vi "Calculate Analog and Digital Channel Values.vi"(8 "Use Default Values":bool=TRUE, 9 "Execute Sequence":bool=TRUE, 10 "current time":timestamp, 11 "Settings in":T1) -> (0 "Digital Values to Write":bool[](array[boolean]), 1 "Analog Values to Write":dbl[](array[numeric]), 2 "Sequence State Channels to Write":dbl[](array[numeric]), 3 "Settings out":T1)   [LabVIEW 2020, in "Sequencer with Output Values.lvlib" / "Sequencer with Output Values.lvclass"]
uses:
  Sequencer with Output Values.lvclass
  Params.ctl
  Step Settings.ctl
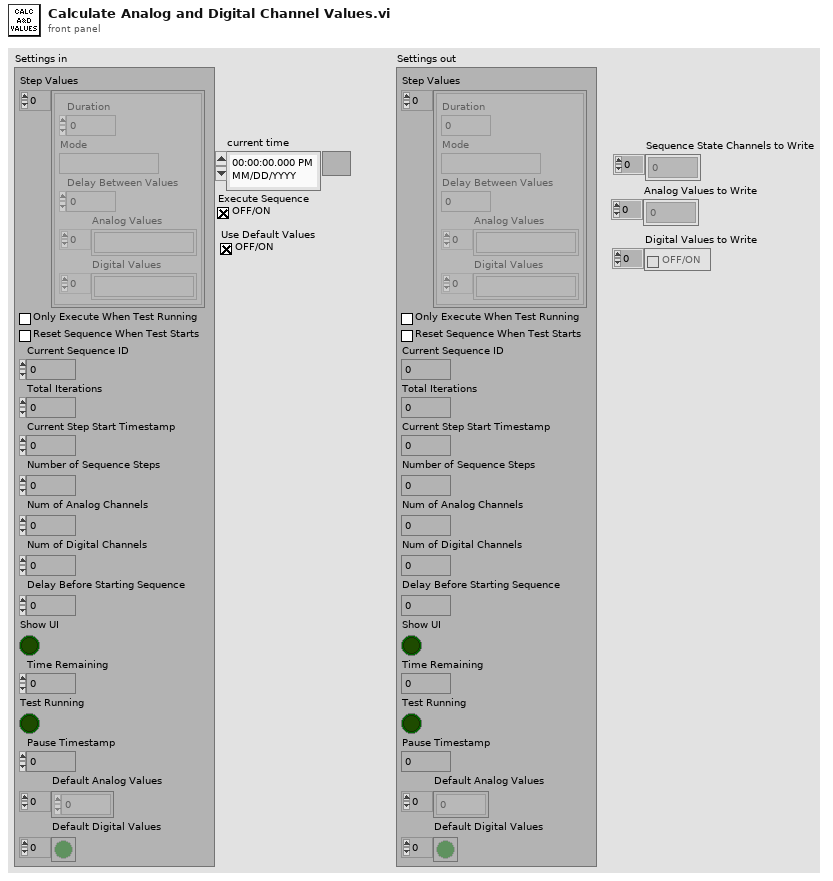
[diagram p1: front panel]
types:
  T1 = typedef "Sequencer with Output Values.lvlib/Sequencer with Output Values.lvclass/Params.ctl" = cluster{"Step Values":T2[], "Only Execute When Test Running":bool, "Reset Sequence When Test Starts":bool, "Current Sequence ID":u32, "Total Iterations":u32, "Current Step Start Timestamp":dbl, "Number of Sequence Steps":i32, "Num of Analog Channels":i32, "Num of Digital Channels":i32, "Delay Before Starting Sequence":dbl, "Show UI":bool, "Time Remaining":dbl, "Test Running":bool, "Pause Timestamp":dbl, "Default Analog Values":dbl[], "Default Digital Values":bool[]}
  T2 = typedef "Sequencer with Output Values.lvlib/Sequencer with Output Values.lvclass/Step Settings.ctl" = cluster{"Duration":dbl, "Mode":string, "Delay Between Values":dbl, "Analog Values":string[], "Digital Values":string[]}
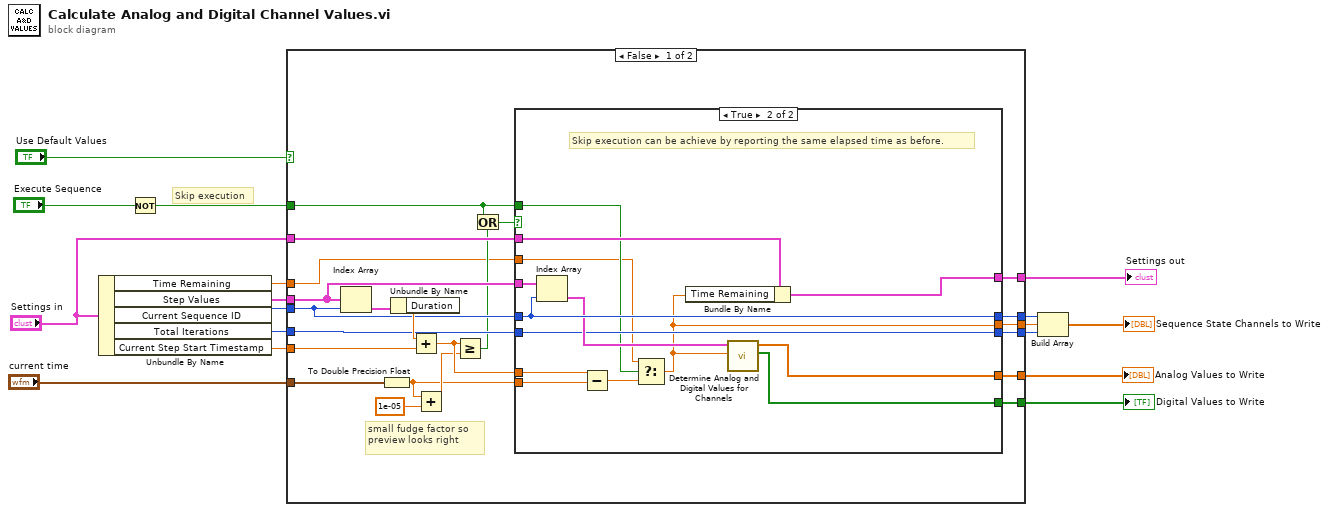
[diagram p0: block diagram]
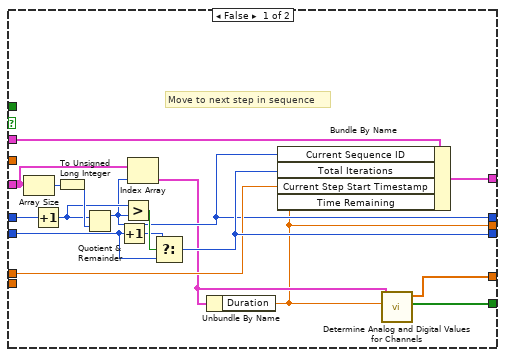
[diagram p2: hidden frame]
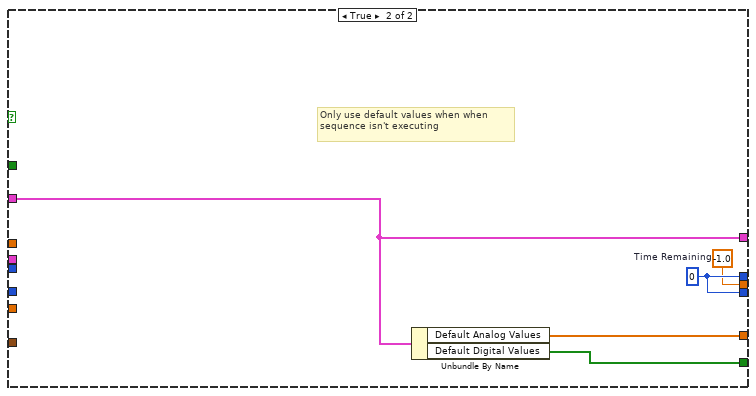
[diagram p3: hidden frame]
diagram:
  # "Skip execution"
  n1 = Unbundle By Name("Settings in") -> ("Time Remaining"=w2:dbl, "Step Values"=w13:T2[], "Current Sequence ID"=w15:u32, "Total Iterations"=w14:u32, "Current Step Start Timestamp"=w16:dbl)
  n2 = Not(x="Execute Sequence") -> (.not. x?=w3:bool)
  n3 = case shown="False" "Use Default Values" {
    tunnel: [w39 w75] -> w17
    tunnel: w16 -> [w35 _]
    tunnel: w15 -> [w34 _]
    tunnel: w14 -> [w33 _]
    tunnel: w13 -> [w32 _]
    tunnel: "current time" -> [w31 _]
    tunnel: [w27 w71] -> w10
    tunnel: [w26 w72] -> w9
    tunnel: [w25 w72] -> w8
    tunnel: [w24 w74] -> w7
    tunnel: [w23 w73] -> w6
    tunnel: "Settings in" -> [w22 w75]
    tunnel: w3 -> [w19 _]
    tunnel: w2 -> [w18 _]
    frame False {
      # "small fudge factor so preview looks right"
      n4 = Index Array(array=w32, index=w34) -> (element=w38:T2)
      n5 = To Double Precision Float(number=w31) -> (double precision float=w28:dbl)
      n6 = Unbundle By Name(w38) -> ("Duration"=w36:dbl)
      n7 = Add(x=w36, y=w35) -> (x+y=w37:dbl)
      n8 = Add(x=w28, y=1e-05) -> (x+y=w29:dbl)
      n9 = Greater Or Equal?(x=w37, y=w29) -> (x >= y?=w21:bool)
      n10 = Or(x=w19, y=w21) -> (x .or. y?=w20:bool)
      n11 = case shown="True" w20 {
        tunnel: w22 -> [w51 w65]
        tunnel: w34 -> [w55 w69]
        tunnel: w32 -> [w45 w70]
        tunnel: w33 -> [w53 w64]
        tunnel: [w44 w69] -> w26
        tunnel: [w49 w64] -> w25
        tunnel: [w50 w63] -> w39
        tunnel: w37 -> [w46 w61]
        tunnel: w28 -> [_ w62]
        tunnel: [w40 w57] -> w27
        tunnel: [w43 w67] -> w24
        tunnel: [w42 w66] -> w23
        tunnel: w19 -> [_ w59]
        tunnel: w18 -> [_ w58]
        frame False {
          # "Move to next step in sequence"
          n12 = Array Size(array=w45) -> (size(s)=w56:i32)
          n13 = Increment(x=w55) -> (x+1=w47:u32)
          n14 = To Unsigned Long Integer(number=w56) -> (unsigned 32bit integer=w48:u32)
          n15 = Quotient & Remainder(x=w47, y=w48) -> (x-y*floor(x/y)=w44:u32)  [unwired: 1 out]
          n16 = Increment(x=w53) -> (x+1=w52:u32)
          n17 = Greater?(x=w47, y=w44) -> (0:w54:bool)
          n18 = Index Array(array=w45, index=w44) -> (element=w41:T2)
          n19 = Select(t=w52, s=w54, f=w53) -> (s? t:f=w49:u32)
          n20 = Unbundle By Name(w41) -> ("Duration"=w40:dbl)
          n21 = Bundle By Name(cluster=w51, "Current Sequence ID"=w44, "Total Iterations"=w49, "Current Step Start Timestamp"=w46, "Time Remaining"=w40) -> (w50:T1)
          n22 = call "Determine Analog and Digital Values for Channels.vi"("Remaining Time"=w40, "Step Settings"=w41) -> ("Digital Values to Write"=w42:bool[], "Analog Values to Write"=w43:dbl[])  [unwired: 8 in]
        }
        frame True {
          # "Skip execution can be achieve by reporting the same elapsed time as before."
          n23 = Index Array(array=w70, index=w69) -> (element=w68:T2)
          n24 = Subtract(x=w61, y=w62) -> (x-y=w60:dbl)
          n25 = Select(t=w58, s=w59, f=w60) -> (s? t:f=w57:dbl)
          n26 = Bundle By Name(cluster=w65, "Time Remaining"=w57) -> (w63:T1)
          n27 = call "Determine Analog and Digital Values for Channels.vi"("Remaining Time"=w57, "Step Settings"=w68) -> ("Digital Values to Write"=w66:bool[], "Analog Values to Write"=w67:dbl[])  [unwired: 8 in]
        }
      }
    }
    frame True {
      w71 = -1.0  # Time Remaining
      w72 = u32 0 ("Current Sequence ID")
      # "Only use default values when when sequence isn't executing"
      n28 = Unbundle By Name(w75) -> ("Default Analog Values"=w74:dbl[], "Default Digital Values"=w73:bool[])
    }
  }
  "Settings out" <- w17
  "Digital Values to Write" <- w6
  "Analog Values to Write" <- w7
  n29 = Build Array(w9, w10, w8) -> (→"Sequence State Channels to Write":dbl[])
